vi "Cmd_Connect.vi"(8 "error in (no error)":errorcluster, 11 "IP myRIO in":string) -> (0 "error out":errorcluster, 1 "connected?":bool, 3 "Refnum out":refnum<k21>)   [LabVIEW 2025]
uses:
  vi/thresholds.ctl
  vi/Command.ctl
  vi/RT_Cmd.ctl
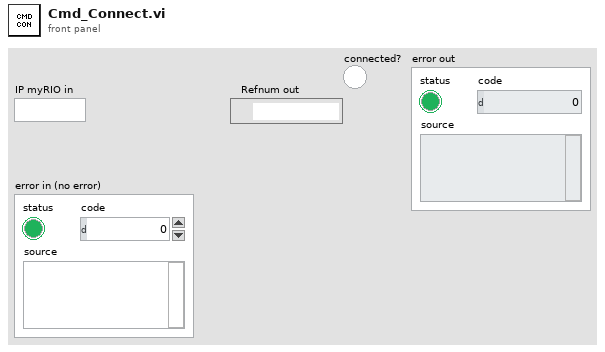
[diagram p1: front panel]
types:
  T1 = typedef "RT_Cmd.ctl" = cluster{"command":T2, "parameters":T3}
  T2 = typedef "Command.ctl" = enum16{"threshold_config", "manual_trigger", "stop"}
  T3 = typedef "thresholds.ctl" = cluster{"Thr_X":i16, "Thr_Y":i16, "Thr_Z":i16}
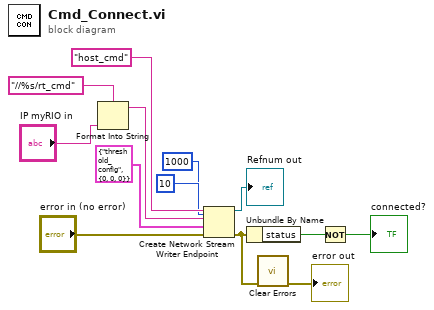
[diagram p0: block diagram]
diagram:
  n1 = Format Into String(format string="//%s/rt_cmd", "IP myRIO in") -> (resulting string=w5:string)  [unwired: 2 in, 1 out]
  n2 = Create Network Stream Writer Endpoint(5:1000 ("timeout in ms (-1)"), 7:10 ("writer buffer size"), 8:"error in (no error)", 9:T1 {"command"=enum."threshold_config", "parameters"={"Thr_X"=0, "Thr_Y"=0, "Thr_Z"=0}} ("data"), 10:w5, 11:"host_cmd" ("writer name")) -> (0:w1:errorcluster, 3:→"Refnum out":refnum<k21>)  [unwired: 1 in]
  n3 = Unbundle By Name(w1) -> ("status"=w4:bool)
  n4 = call <vilib>:"Clear Errors.vi"("error in (no error)"=w1) -> ("error out"=→"error out":errorcluster)  [unwired: 5 in, 1 out]
  n5 = Not(x=w4) -> (.not. x?=→"connected?":bool)
